vi "draw.notes.vi"(8 "error in (no error)":errorcluster, 11 "midi-ui in":refnum<class "midi-ui.lvclass">) -> (0 "error out":errorcluster, 3 "midi-ui out":refnum<class "midi-ui.lvclass">)   [LabVIEW 2020, in "midi-ui.lvclass"]
uses:
  midi-ui.lvclass
  shared/midi note number.ctl
  midi-ui.lvclass/midi-ui.ctl
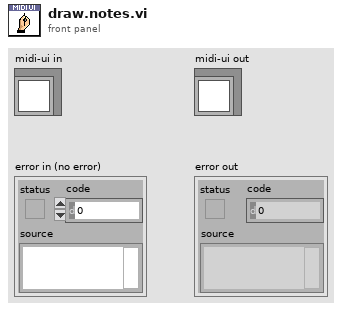
[diagram p1: front panel]
types:
  T1 = typedef "midi note number.ctl" = enum8{"0 - C-1 - 8.18", "1 - C#-1 - 8.66", "2 - D-1 - 9.18", "3 - D#-1 - 9.72", "4 - E-1 - 10.30", "5 - F-1 - 10.91", "6 - F#-1 - 11.56", "7 - G-1 - 12.25", "8 - G#-1 - 12.98", "9 - A-1 - 13.75", "10 - A#-1 - 14.57", "11 - B-1 - 15.43", "12 - C0 - 16.35", "13 - C#0 - 17.32", "14 - D0 - 18.35", "15 - D#0 - 19.45", "16 - E0 - 20.60", "17 - F0 - 21.83", "18 - F#0 - 23.12", "19 - G0 - 24.50", "20 - G#0 - 25.96", "21 - A0 - 27.50", "22 - A#0 - 29.14", "23 - B0 - 30.87", "24 - C1 - 32.70", "25 - C#1 - 34.65", "26 - D1 - 36.71", "27 - D#1 - 38.89", "28 - E1 - 41.20", "29 - F1 - 43.65", "30 - F#1 - 46.25", "31 - G1 - 49.00", "32 - G#1 - 51.91", "33 - A1 - 55.00", "34 - A#1 - 58.27", "35 - B1 - 61.74", "36 - C2 - 65.41", "37 - C#2 - 69.30", "38 - D2 - 73.42", "39 - D#2 - 77.78", "40 - E2 - 82.41", "41 - F2 - 87.31", "42 - F#2 - 92.50", "43 - G2 - 98.00", "44 - G#2 - 103.83", "45 - A2 - 110.00", "46 - A#2 - 116.54", "47 - B2 - 123.47", "48 - C3 - 130.81", "49 - C#3 - 138.59", "50 - D3 - 146.83", "51 - D#3 - 155.56", "52 - E3 - 164.81", "53 - F3 - 174.61", "54 - F#3 - 185.00", "55 - G3 - 196.00", "56 - G#3 - 207.65", "57 - A3 - 220.00", "58 - A#3 - 233.08", "59 - B3 - 246.94", "60 - C4 - 261.63", "61 - C#4 - 277.18", "62 - D4 - 293.66", "63 - D#4 - 311.13", "64 - E4 - 329.63", "65 - F4 - 349.23", "66 - F#4 - 369.99", "67 - G4 - 392.00", "68 - G#4 - 415.30", "69 - A4 - 440.00", "70 - A#4 - 466.16", "71 - B4 - 493.88", "72 - C5 - 523.25", "73 - C#5 - 554.37", "74 - D5 - 587.33", "75 - D#5 - 622.25", "76 - E5 - 659.25", "77 - F5 - 698.46", "78 - F#5 - 739.99", "79 - G5 - 783.99", "80 - G#5 - 830.61", "81 - A5 - 880.00", "82 - A#5 - 932.33", "83 - B5 - 987.77", "84 - C6 - 1046.50", "85 - C#6 - 1108.73", "86 - D6 - 1174.66", "87 - D#6 - 1244.51", "88 - E6 - 1318.51", "89 - F6 - 1396.91", "90 - F#6 - 1479.98", "91 - G6 - 1567.98", "92 - G#6 - 1661.22", "93 - A6 - 1760.00", "94 - A#6 - 1864.66", "95 - B6 - 1975.53", "96 - C7 - 2093.00", "97 - C#7 - 2217.46", "98 - D7 - 2349.32", "99 - D#7 - 2489.02", "100 - E7 - 2637.02", "101 - F7 - 2793.83", "102 - F#7 - 2959.96", "103 - G7 - 3135.96", "104 - G#7 - 3322.44", "105 - A7 - 3520.00", "106 - A#7 - 3729.31", "107 - B7 - 3951.07", "108 - C8 - 4186.01", "109 - C#8 - 4434.92", "110 - D8 - 4698.63", "111 - D#8 - 4978.03", "112 - E8 - 5274.04", "113 - F8 - 5587.65", "114 - F#8 - 5919.91", "115 - G8 - 6271.93", "116 - G#8 - 6644.88", "117 - A8 - 7040.00", "118 - A#8 - 7458.62", "119 - B8 - 7902.13", "120 - C9 - 8372.02", "121 - C#9 - 8869.84", "122 - D9 - 9397.27", "123 - D#9 - 9956.06", "124 - E9 - 10548.08", "125 - F9 - 11175.30", "126 - F#9 - 11839.82", "127 - G9 - 12543.85"}
  T2 = map{T1, cluster{"Note On":picture, "Note Off":picture}}
  T3 = typedef "midi-ui.lvclass/privatedata.ctl" = cluster{"White Key Length":dbl, "White Key Width":dbl, "Black Key Length":dbl, "Key Polygon Corners by Name":map{string, cluster{"x":dbl, "y":dbl}[]}, "Anticlockwise rotations [0-3] (0)":i32, "Polygon Corners by Note Name":map{T1, cluster{"x":dbl, "y":dbl}[]}, "Picture Control":refnum<vi>, "Owning VI":refnum<vi>, "Control Index":i32, "Keyboard Key Note Bounds by Note Name":map{T1, cluster{"max":dbl, "min":dbl}}, "Notes on screen":cluster{"Note":T1, "End Time":u32, "Start Time":u32}[], "Polygon Pictures by Note Name":map{T1, cluster{"Note On":picture, "Note Off":picture}}, "keyboard":picture[], "Keyboard Note Picture Index by Name":map{T1, i32}, "music":picture[], "Zoom Factor":sgl, "keyboard - all off":picture[]}
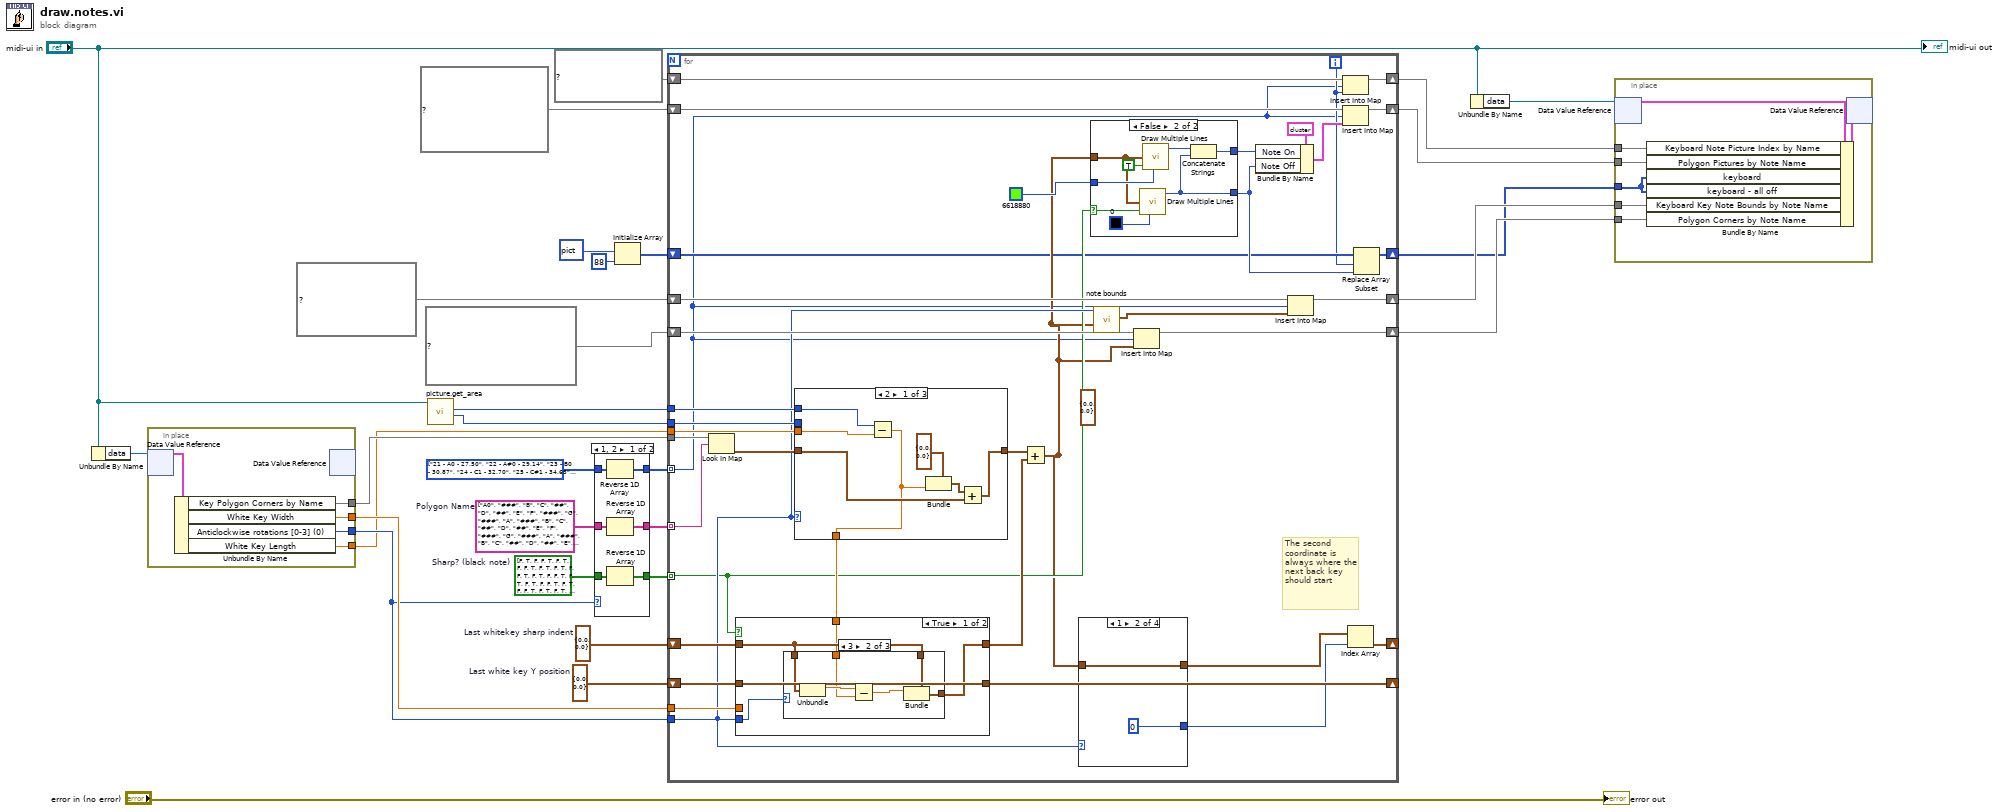
[diagram p0: block diagram]
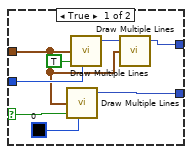
[diagram p3: hidden frame]
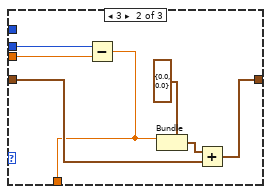
[diagram p4: hidden frame]
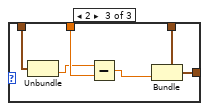
[diagram p7: hidden frame]
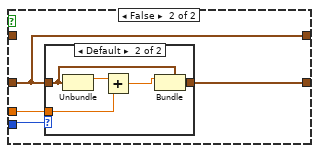
[diagram p8: hidden frame]
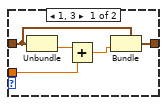
[diagram p9: hidden frame]
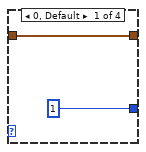
[diagram p10: hidden frame]
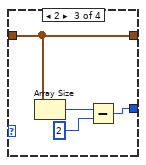
[diagram p11: hidden frame]
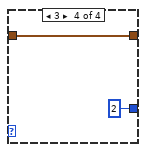
[diagram p12: hidden frame]
diagram:
  w3 = T1[] [enum."21 - A0 - 27.50", enum."22 - A#0 - 29.14", enum."23 - B0 - 30.87", enum."24 - C1 - 32.70", enum."25 - C#1 - 34.65", enum."26 - D1 - 36.71", enum."27 - D#1 - 38.89", enum."28 - E1 - 41.20", enum."29 - F1 - 43.65", enum."30 - F#1 - 46.25", enum."31 - G1 - 49.00", enum."32 - G#1 - 51.91", enum."33 - A1 - 55.00", enum."34 - A#1 - 58.27", enum."35 - B1 - 61.74", enum."36 - C2 - 65.41", enum."37 - C#2 - 69.30", enum."38 - D2 - 73.42", enum."39 - D#2 - 77.78", enum."40 - E2 - 82.41", enum."41 - F2 - 87.31", enum."42 - F#2 - 92.50", enum."43 - G2 - 98.00", enum."44 - G#2 - 103.83", enum."45 - A2 - 110.00", enum."46 - A#2 - 116.54", enum."47 - B2 - 123.47", enum."48 - C3 - 130.81", enum."49 - C#3 - 138.59", enum."50 - D3 - 146.83", enum."51 - D#3 - 155.56", enum."52 - E3 - 164.81", enum."53 - F3 - 174.61", enum."54 - F#3 - 185.00", enum."55 - G3 - 196.00", enum."56 - G#3 - 207.65", enum."57 - A3 - 220.00", enum."58 - A#3 - 233.08", enum."59 - B3 - 246.94", enum."60 - C4 - 261.63", enum."61 - C#4 - 277.18", enum."62 - D4 - 293.66", enum."63 - D#4 - 311.13", enum."64 - E4 - 329.63", enum."65 - F4 - 349.23", enum."66 - F#4 - 369.99", enum."67 - G4 - 392.00", enum."68 - G#4 - 415.30", enum."69 - A4 - 440.00", enum."70 - A#4 - 466.16", enum."71 - B4 - 493.88", enum."72 - C5 - 523.25", enum."73 - C#5 - 554.37", enum."74 - D5 - 587.33", enum."75 - D#5 - 622.25", enum."76 - E5 - 659.25", enum."77 - F5 - 698.46", enum."78 - F#5 - 739.99", enum."79 - G5 - 783.99", enum."80 - G#5 - 830.61", enum."81 - A5 - 880.00", enum."82 - A#5 - 932.33", enum."83 - B5 - 987.77", enum."84 - C6 - 1046.50", enum."85 - C#6 - 1108.73", enum."86 - D6 - 1174.66", enum."87 - D#6 - 1244.51", enum."88 - E6 - 1318.51", enum."89 - F6 - 1396.91", enum."90 - F#6 - 1479.98", enum."91 - G6 - 1567.98", enum."92 - G#6 - 1661.22", enum."93 - A6 - 1760.00", enum."94 - A#6 - 1864.66", enum."95 - B6 - 1975.53", enum."96 - C7 - 2093.00", enum."97 - C#7 - 2217.46", enum."98 - D7 - 2349.32", enum."99 - D#7 - 2489.02", enum."100 - E7 - 2637.02", enum."101 - F7 - 2793.83", enum."102 - F#7 - 2959.96", enum."103 - G7 - 3135.96", enum."104 - G#7 - 3322.44", enum."105 - A7 - 3520.00", enum."106 - A#7 - 3729.31", enum."107 - B7 - 3951.07", enum."108 - C8 - 4186.01"] items=["0 - C-1 - 8.18", "1 - C#-1 - 8.66", "2 - D-1 - 9.18", "3 - D#-1 - 9.72", "4 - E-1 - 10.30", "5 - F-1 - 10.91", "6 - F#-1 - 11.56", "7 - G-1 - 12.25", "8 - G#-1 - 12.98", "9 - A-1 - 13.75", "10 - A#-1 - 14.57", "11 - B-1 - 15.43", "12 - C0 - 16.35", "13 - C#0 - 17.32", "14 - D0 - 18.35", "15 - D#0 - 19.45", "16 - E0 - 20.60", "17 - F0 - 21.83", "18 - F#0 - 23.12", "19 - G0 - 24.50", "20 - G#0 - 25.96", "21 - A0 - 27.50", "22 - A#0 - 29.14", "23 - B0 - 30.87", "24 - C1 - 32.70", "25 - C#1 - 34.65", "26 - D1 - 36.71", "27 - D#1 - 38.89", "28 - E1 - 41.20", "29 - F1 - 43.65", "30 - F#1 - 46.25", "31 - G1 - 49.00", "32 - G#1 - 51.91", "33 - A1 - 55.00", "34 - A#1 - 58.27", "35 - B1 - 61.74", "36 - C2 - 65.41", "37 - C#2 - 69.30", "38 - D2 - 73.42", "39 - D#2 - 77.78", "40 - E2 - 82.41", "41 - F2 - 87.31", "42 - F#2 - 92.50", "43 - G2 - 98.00", "44 - G#2 - 103.83", "45 - A2 - 110.00", "46 - A#2 - 116.54", "47 - B2 - 123.47", "48 - C3 - 130.81", "49 - C#3 - 138.59", "50 - D3 - 146.83", "51 - D#3 - 155.56", "52 - E3 - 164.81", "53 - F3 - 174.61", "54 - F#3 - 185.00", "55 - G3 - 196.00", "56 - G#3 - 207.65", "57 - A3 - 220.00", "58 - A#3 - 233.08", "59 - B3 - 246.94", "60 - C4 - 261.63", "61 - C#4 - 277.18", "62 - D4 - 293.66", "63 - D#4 - 311.13", "64 - E4 - 329.63", "65 - F4 - 349.23", "66 - F#4 - 369.99", "67 - G4 - 392.00", "68 - G#4 - 415.30", "69 - A4 - 440.00", "70 - A#4 - 466.16", "71 - B4 - 493.88", "72 - C5 - 523.25", "73 - C#5 - 554.37", "74 - D5 - 587.33", "75 - D#5 - 622.25", "76 - E5 - 659.25", "77 - F5 - 698.46", "78 - F#5 - 739.99", "79 - G5 - 783.99", "80 - G#5 - 830.61", "81 - A5 - 880.00", "82 - A#5 - 932.33", "83 - B5 - 987.77", "84 - C6 - 1046.50", "85 - C#6 - 1108.73", "86 - D6 - 1174.66", "87 - D#6 - 1244.51", "88 - E6 - 1318.51", "89 - F6 - 1396.91", "90 - F#6 - 1479.98", "91 - G6 - 1567.98", "92 - G#6 - 1661.22", "93 - A6 - 1760.00", "94 - A#6 - 1864.66", "95 - B6 - 1975.53", "96 - C7 - 2093.00", "97 - C#7 - 2217.46", "98 - D7 - 2349.32", "99 - D#7 - 2489.02", "100 - E7 - 2637.02", "101 - F7 - 2793.83", "102 - F#7 - 2959.96", "103 - G7 - 3135.96", "104 - G#7 - 3322.44", "105 - A7 - 3520.00", "106 - A#7 - 3729.31", "107 - B7 - 3951.07", "108 - C8 - 4186.01", "109 - C#8 - 4434.92", "110 - D8 - 4698.63", "111 - D#8 - 4978.03", "112 - E8 - 5274.04", "113 - F8 - 5587.65", "114 - F#8 - 5919.91", "115 - G8 - 6271.93", "116 - G#8 - 6644.88", "117 - A8 - 7040.00", "118 - A#8 - 7458.62", "119 - B8 - 7902.13", "120 - C9 - 8372.02", "121 - C#9 - 8869.84", "122 - D9 - 9397.27", "123 - D#9 - 9956.06", "124 - E9 - 10548.08", "125 - F9 - 11175.30", "126 - F#9 - 11839.82", "127 - G9 - 12543.85"] ("Array")
  w26 = bool[] [FALSE, TRUE, FALSE, FALSE, TRUE, FALSE, TRUE, FALSE, FALSE, TRUE, FALSE, TRUE, FALSE, TRUE, FALSE, FALSE, TRUE, FALSE, TRUE, FALSE, FALSE, TRUE, FALSE, TRUE, FALSE, TRUE, FALSE, FALSE, TRUE, FALSE, TRUE, FALSE, FALSE, TRUE, FALSE, TRUE, FALSE, TRUE, FALSE, FALSE, TRUE, FALSE, TRUE, FALSE, FALSE, TRUE, FALSE, TRUE, FALSE, TRUE, FALSE, FALSE, TRUE, FALSE, TRUE, FALSE, FALSE, TRUE, FALSE, TRUE, FALSE, TRUE, FALSE, FALSE, TRUE, FALSE, TRUE, FALSE, FALSE, TRUE, FALSE, TRUE, FALSE, TRUE, FALSE, FALSE, TRUE, FALSE, TRUE, FALSE, FALSE, TRUE, FALSE, TRUE, FALSE, TRUE, FALSE, FALSE]  # Sharp? (black note)
  w27 = string[] ["A0", "###", "B", "C", "##", "D", "##", "E", "F", "###", "G", "###", "A", "###", "B", "C", "##", "D", "##", "E", "F", "###", "G", "###", "A", "###", "B", "C", "##", "D", "##", "E", "F", "###", "G", "###", "A", "###", "B", "C", "##", "D", "##", "E", "F", "###", "G", "###", "A", "###", "B", "C", "##", "D", "##", "E", "F", "###", "G", "###", "A", "###", "B", "C", "##", "D", "##", "E", "F", "###", "G", "###", "A", "###", "B", "C", "##", "D", "##", "E", "F", "###", "G", "###", "A", "###", "B", "C8"]  # Polygon Name
  w29 = cluster{"x":dbl, "y":dbl} {"x"=0.0, "y"=0.0}  # Last whitekey sharp indent
  w30 = cluster{"x":dbl, "y":dbl} {"x"=0.0, "y"=0.0}  # Last white key Y position
  n1 = Unbundle By Name("midi-ui in") -> ("data"=w16:refnum<data-value>)
  n2 = in-place {
    in-place-border: [w34] -> w15
    in-place-border: [w33] -> w14
    in-place-border: [w32] -> w13
    in-place-border: [w31] -> w12
    n3 = in-place-dvr #1(w16) -> (w35:T3)  [unwired: 1 out]
    n4 = Unbundle By Name(w35) -> ("Key Polygon Corners by Name"=w34:map{string, cluster{"x":dbl, "y":dbl}[]}, "White Key Width"=w33:dbl, "Anticlockwise rotations [0-3] (0)"=w32:i32, "White Key Length"=w31:dbl)
    n5 = in-place-dvr #1() -> ()  [unwired: 1 in, 2 out]
  }
  n6 = call "picture.get_area.vi"("midi-ui in"="midi-ui in") -> ("Bounds:Area Width"=w17:u32, "Bounds:Area Height"=w18:u32)  [unwired: 7 in, 2 out]
  n7 = case shown="1, 2" w13 {
    tunnel: w3 -> [w41 w44]
    tunnel: w27 -> [w40 w43]
    tunnel: w26 -> [w39 w42]
    tunnel: [w38 w44] -> w25
    tunnel: [w37 w43] -> w24
    tunnel: [w36 w42] -> w23
    frame 1, 2 {
      n8 = Reverse 1D Array(array=w41) -> (reversed array=w38:T1[])
      n9 = Reverse 1D Array(array=w40) -> (reversed array=w37:string[])
      n10 = Reverse 1D Array(array=w39) -> (reversed array=w36:bool[])
    }
    frame Default {
    }
  }
  n11 = Initialize Array(picture data[5B] ("new picture"), 88 ("dimension size")) -> (w6:picture[])
  n12 = for {
    tunnel: w15 -> [w81]
    tunnel: w25 -> [w45] mode=indexing
    shift-right: [w80] -> _
    shift-left: w30 -> [w79]
    shift-right: [w76] -> _
    shift-left: w29 -> [w77]
    shift-right: [w50] -> w11
    shift-left: map{T1, cluster{"max":dbl, "min":dbl}[]} {} ("Note Bounds by Note Name") -> [w75]
    tunnel: w24 -> [w74] mode=indexing
    tunnel: w23 -> [w55] mode=indexing
    tunnel: w14 -> [w73]
    tunnel: w13 -> [w61]
    tunnel: w18 -> [w70]
    tunnel: w12 -> [w69]
    tunnel: w17 -> [w68]
    shift-right: [w63] -> w10
    shift-left: map{T1, cluster{"max":dbl, "min":dbl}} {} ("Note Bounds by Note Name") -> [w64]
    shift-right: [w60] -> w2
    shift-left: T2 {} ("Polygon Pictures by Note Name") -> [w59]
    shift-right: [w53] -> w9
    shift-left: map{T1, i32} {} ("Keyboard Note Index by Name") -> [w54]
    shift-right: [w49] -> w1
    shift-left: w6 -> [w47]
    i -> [w46]
    (unwired) cluster{"max":dbl, "min":dbl} {"max"=0.0, "min"=0.0} ("value")
    # "The second coordinate is always where the next back key should start"
    n13 = Look In Map(map=w81, key=w74) -> (value=w66:cluster{"x":dbl, "y":dbl}[])  [unwired: 1 in, 1 out]
    n14 = case shown="2" w61 {
      tunnel: [w99 w107 w112] -> w71
      tunnel: w66 -> [w101 w109 w112]
      tunnel: w70 -> [w104 _ _]
      tunnel: w69 -> [w103 w111 _]
      tunnel: w68 -> [_ w106 _]
      tunnel: [w98 w105 _] -> w65
      frame 2 {
        n15 = Subtract(x=w104, y=w103) -> (x-y=w98:dbl)
        n16 = Bundle(cluster=cluster{"x":dbl, "y":dbl} {"x"=0.0, "y"=0.0} ("coordinate"), "y"=w98) -> (w102:cluster{"x":dbl, "y":dbl})  [unwired: 1 in]
        n17 = Add(x=w102, y=w101) -> (x+y=w99:cluster{"x":dbl, "y":dbl}[])
      }
      frame 3 {
        n18 = Subtract(x=w106, y=w111) -> (x-y=w105:dbl)
        n19 = Bundle(cluster=cluster{"x":dbl, "y":dbl} {"x"=0.0, "y"=0.0} ("coordinate"), "x"=w105) -> (w110:cluster{"x":dbl, "y":dbl})  [unwired: 1 in]
        n20 = Add(x=w110, y=w109) -> (x+y=w107:cluster{"x":dbl, "y":dbl}[])
      }
      frame Default {
      }
    }
    n21 = case shown="True" w55 {
      tunnel: w79 -> [w117 w133]
      tunnel: [w117 w134] -> w80
      tunnel: [w115 w133] -> w78
      tunnel: w77 -> [w114 _]
      tunnel: w73 -> [_ w132]
      tunnel: w61 -> [w116 w131]
      tunnel: w65 -> [w113 _]
      frame True {
        n22 = case shown="3" w116 {
          tunnel: w114 -> [w118 w124 w130]
          tunnel: [w118 w123 w129] -> w115
          tunnel: w114 -> [_ w122 w128]
          tunnel: w113 -> [_ w119 w127]
          frame 0, Default {
          }
          frame 3 {
            n23 = Unbundle(w122) -> ("x"=w121:dbl)  [unwired: 1 out]
            n24 = Subtract(x=w121, y=w119) -> (x-y=w120:dbl)
            n25 = Bundle(cluster=w124, "x"=w120) -> (w123:cluster{"x":dbl, "y":dbl})  [unwired: 1 in]
          }
          frame 2 {
            n26 = Unbundle(w128) -> ("y"=w126:dbl)  [unwired: 1 out]
            n27 = Subtract(x=w126, y=w127) -> (x-y=w125:dbl)
            n28 = Bundle(cluster=w130, "y"=w125) -> (w129:cluster{"x":dbl, "y":dbl})  [unwired: 1 in]
          }
        }
      }
      frame False {
        n29 = case shown="Default" w131 {
          tunnel: [w139 w144] -> w134
          tunnel: w133 -> [w137 w140]
          tunnel: w132 -> [w138 w143]
          frame 1, 3 {
            n30 = Unbundle(w137) -> ("y"=w136:dbl)  [unwired: 1 out]
            n31 = Add(x=w136, y=w138) -> (x+y=w135:dbl)
            n32 = Bundle(cluster=w137, "y"=w135) -> (w139:cluster{"x":dbl, "y":dbl})  [unwired: 1 in]
          }
          frame Default {
            n33 = Unbundle(w140) -> ("x"=w142:dbl)  [unwired: 1 out]
            n34 = Add(x=w142, y=w143) -> (x+y=w141:dbl)
            n35 = Bundle(cluster=w140, "x"=w141) -> (w144:cluster{"x":dbl, "y":dbl})  [unwired: 1 in]
          }
        }
      }
    }
    n36 = Add(x=w71, y=w78) -> (x+y=w51:cluster{"x":dbl, "y":dbl}[])
    n37 = case shown="1" w61 {
      tunnel: [1 0 w149 2] -> w72
      tunnel: [w145 w147 w152 w153] -> w67
      tunnel: w51 -> [w145 w147 w152 w153]
      frame 0, Default {
      }
      frame 1 {
      }
      frame 2 {
        n38 = Array Size(array=w152) -> (size(s)=w151:i32)
        n39 = Subtract(x=w151, y=2) -> (x-y=w149:i32)
      }
      frame 3 {
      }
    }
    n40 = case shown="False" w55 {
      selector: w55 -> [w86 w95]
      tunnel: w51 -> [w82 w93]
      tunnel: u32 6618880 ("color(black)") -> [w89 w97]
      tunnel: [w83 w90] -> w52
      tunnel: [w88 w91] -> w48
      frame True {
        n41 = call <vilib>:"Draw Multiple Lines.vi"("line endpoints"=w82, "fill?(F)"=w86, "color(black)"=u32 0) -> ("new picture"=w88:picture)  [unwired: 6 in]
        n42 = call <vilib>:"Draw Multiple Lines.vi"("line endpoints"=w82, "fill?(F)"=TRUE, "color(black)"=w89) -> ("new picture"=w84:picture)  [unwired: 6 in]
        n43 = call <vilib>:"Draw Multiple Lines.vi"("picture"=w84, "line endpoints"=w82) -> ("new picture"=w83:picture)  [unwired: 7 in]
      }
      frame False {
        n44 = call <vilib>:"Draw Multiple Lines.vi"("line endpoints"=w93, "fill?(F)"=w95, "color(black)"=u32 0) -> ("new picture"=w91:picture)  [unwired: 6 in]
        n45 = call <vilib>:"Draw Multiple Lines.vi"("line endpoints"=w93, "fill?(F)"=TRUE, "color(black)"=w97) -> ("new picture"=w92:picture)  [unwired: 6 in]
        n46 = Concatenate Strings(w92, w91) -> (w90:picture)
      }
    }
    n47 = call "note bounds.vi"("Note Polygon"=w51, "Anticlockwise rotations [0-3] (0)"=w61) -> ("Bounds"=w62:cluster{"Max":i16, "Min":i16})  [unwired: 9 in]
    n48 = Insert Into Map(map in=w75, key=w45, value=w51) -> (map out=w50:map{T1, cluster{"max":dbl, "min":dbl}[]})  [unwired: 2 out]
    n49 = Bundle By Name(cluster=cluster{"Note On":picture, "Note Off":picture} {"Note On"=bytes[0], "Note Off"=bytes[0]} ("value"), "Note On"=w52, "Note Off"=w48) -> (w56:cluster{"Note On":picture, "Note Off":picture})
    n50 = Insert Into Map(map in=w64, key=w45, value=w62) -> (map out=w63:map{T1, cluster{"max":dbl, "min":dbl}})  [unwired: 2 out]
    n51 = Insert Into Map(map in=w54, key=w45, value=w46) -> (map out=w53:map{T1, i32})  [unwired: 2 out]
    n52 = Insert Into Map(map in=w59, key=w45, value=w56) -> (map out=w60:T2)  [unwired: 2 out]
    n53 = Index Array(array=w67, index=w72) -> (element=w76:cluster{"x":dbl, "y":dbl})
    n54 = Replace Array Subset(array=w47, new element=w48, index=w46) -> (w49:picture[])
  }
  n55 = Unbundle By Name("midi-ui in") -> ("data"=w5:refnum<data-value>)
  n56 = in-place {
    in-place-border: w11 -> [w159]
    in-place-border: w10 -> [w158]
    in-place-border: w2 -> [w156]
    in-place-border: w9 -> [w157]
    in-place-border: w1 -> [w155]
    n57 = in-place-dvr #2(w5) -> (w161:T3)  [unwired: 1 out]
    n58 = Bundle By Name(cluster=w161, "Keyboard Note Picture Index by Name"=w157, "Polygon Pictures by Note Name"=w156, "keyboard"=w155, "keyboard - all off"=w155, "Keyboard Key Note Bounds by Note Name"=w158, "Polygon Corners by Note Name"=w159) -> (w160:T3)
    n59 = in-place-dvr #2(w160) -> ()  [unwired: 2 out]
  }
  "error out" <- "error in (no error)"
  "midi-ui out" <- "midi-ui in"
